vi "Write Debug info.vi"(9 "Debug info":string, 11 "CDebugInfo in":refnum<class "CDebugInfo.lvclass">) -> (3 "CDebugInfo out":refnum<class "CDebugInfo.lvclass">)   [LabVIEW 2020, in "DependencyInspection.lvlib" / "CDebugInfo.lvclass"]
uses:
  CDebugInfo.lvclass
  CDebugInfo.lvclass/CDebugInfo.ctl
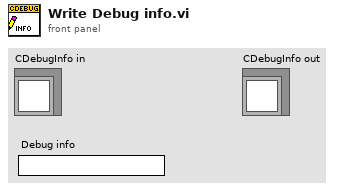
[diagram p1: front panel]
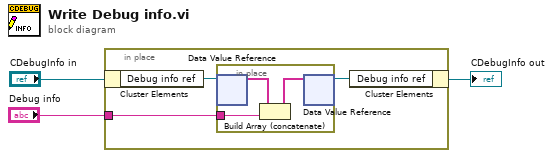
[diagram p0: block diagram]
diagram:
  n1 = in-place {
    in-place-border: "Debug info" -> [w6]
    n2 = in-place-cluster #1("CDebugInfo in") -> ("Debug info ref"=w5:refnum<data-value>)
    n3 = in-place {
      in-place-border: w6 -> [w9]
      n4 = in-place-dvr #2(w5) -> (w8:string[])  [unwired: 1 out]
      n5 = Build Array (concatenate)(w8, w9) -> (w7:string[])
      n6 = in-place-dvr #2(w7) -> (w4:refnum<data-value>)  [unwired: 1 out]
    }
    n7 = in-place-cluster #1("Debug info ref"=w4) -> (→"CDebugInfo out":refnum<class "CDebugInfo.lvclass">)
  }
